vi "Test_INL.vi"(0 "Value":refnum<vi>, 5 "Total":refnum<vi>, 11 "Error In":errorcluster) -> (4 "INL":dbl[](array[numeric]) format="%#.6g", 6 "Codes Array":i32[](array[numeric]), 15 "Error Out":errorcluster)   [LabVIEW 2026, in "Core.lvlib"]
doc: "Calculates INL values and identifies the corresponding converter codes for linearity characterization."
uses:
  Core.lvlib
  TypeDefs/Enum_Notifier_Name.ctl
  TypeDefs/Enum_Notifier_Options.ctl
  TypeDefs/Notification_Clusters/Cluster_INL_Measurement_Specs.ctl
  <instrlib>/niDCPower/nidcpower.llb/niDCPower Output Function.ctl
  TypeDefs/Notification_Clusters/Cluster_ADC_Instrument_Specs.ctl
  TypeDefs/Notification_Clusters/Cluster_DAC_Instrument_Specs.ctl
  <instrlib>/niDCPower/nidcpower.llb/niDCPower Measurement Type.ctl
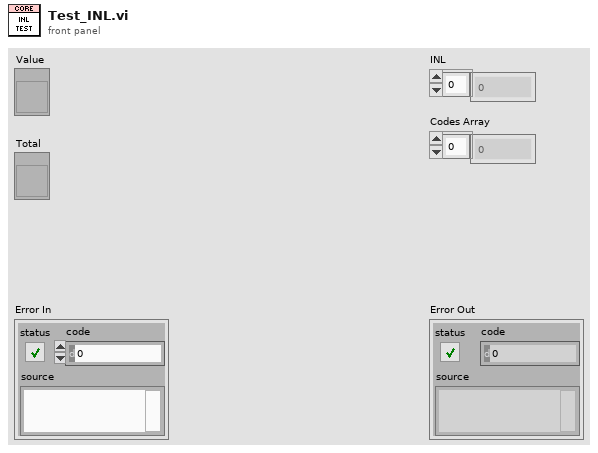
[diagram p1: front panel]
types:
  T1 = typedef "Core.lvlib/Cluster_INL_Measurement_Specs.ctl" = cluster{" Resolution":u16, "Reference Voltage":dbl, "Settling Time (ms)":u32, "Start":dbl, "Step Size":dbl, "Stop":dbl}
  T2 = typedef "Core.lvlib/Enum_Notifier_Options.ctl" = enum16{"Create", "Send", "Status", "Release"}
  T3 = typedef "Core.lvlib/Enum_Notifier_Name.ctl" = enum16{"Device Type", "Test", "Instrument Spec", "Measurement Spec", "Status"}
  T4 = typedef "Core.lvlib/Cluster_ADC_Instrument_Specs.ctl" = cluster{"ADC Source":refnum<k15>, "Current Limit":dbl, "Voltage Level Range":dbl, "ADC DUT":string}
  T5 = typedef "Core.lvlib/Cluster_DAC_Instrument_Specs.ctl" = cluster{"DAC Measurement Device":refnum<k15>, "Current Limit":dbl, "Voltage Level Range":dbl, "DAC DUT":string}
  T6 = typedef "niDCPower Output Function.ctl" = i32
  T7 = typedef "niDCPower Measurement Type.ctl" = i32
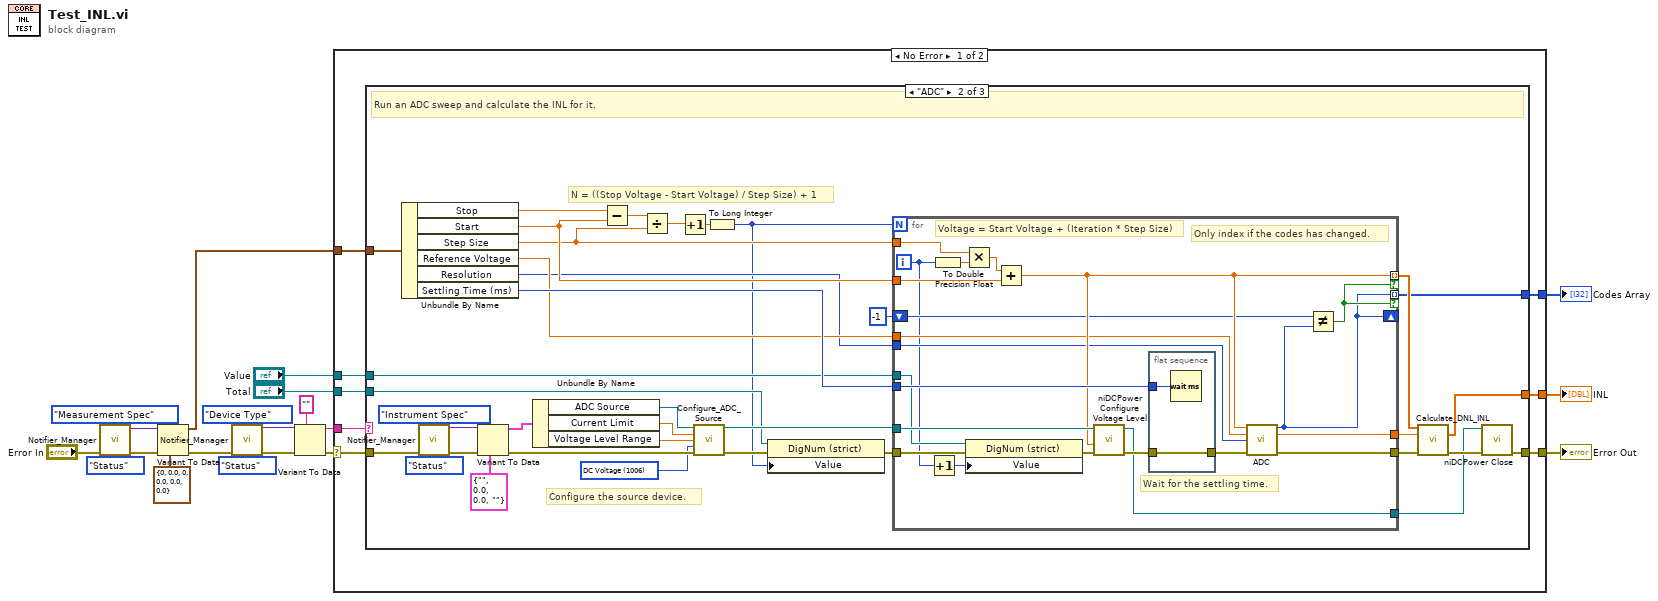
[diagram p0: block diagram]
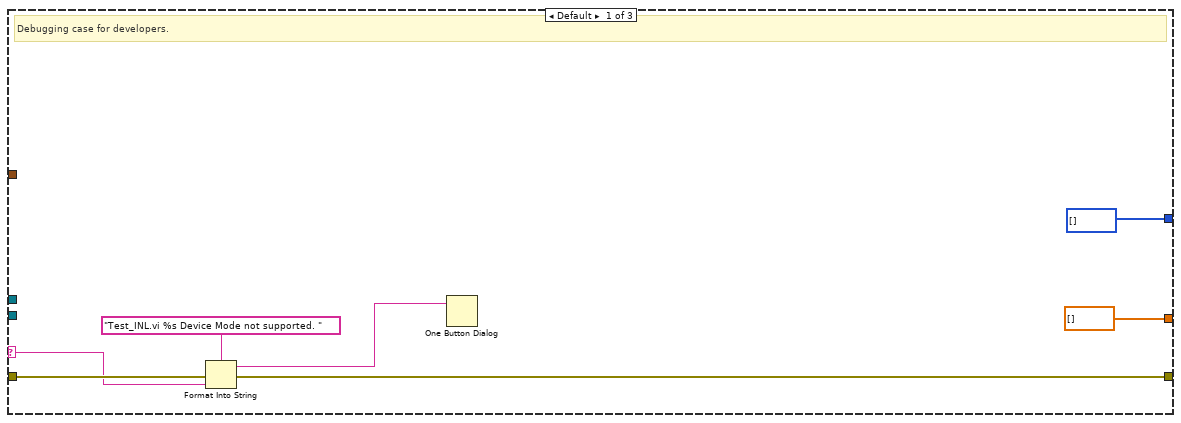
[diagram p2: hidden frame]
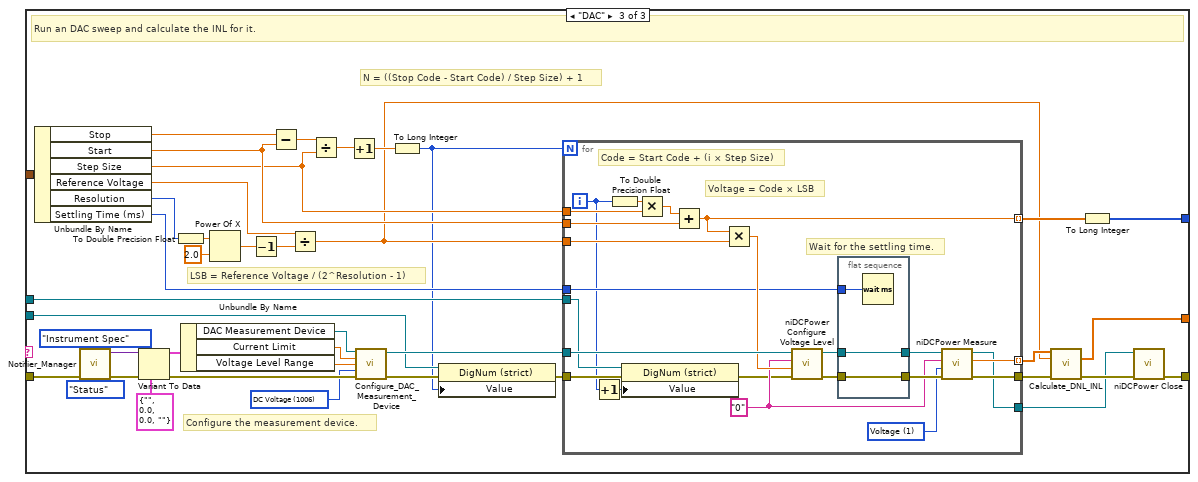
[diagram p3: hidden frame]
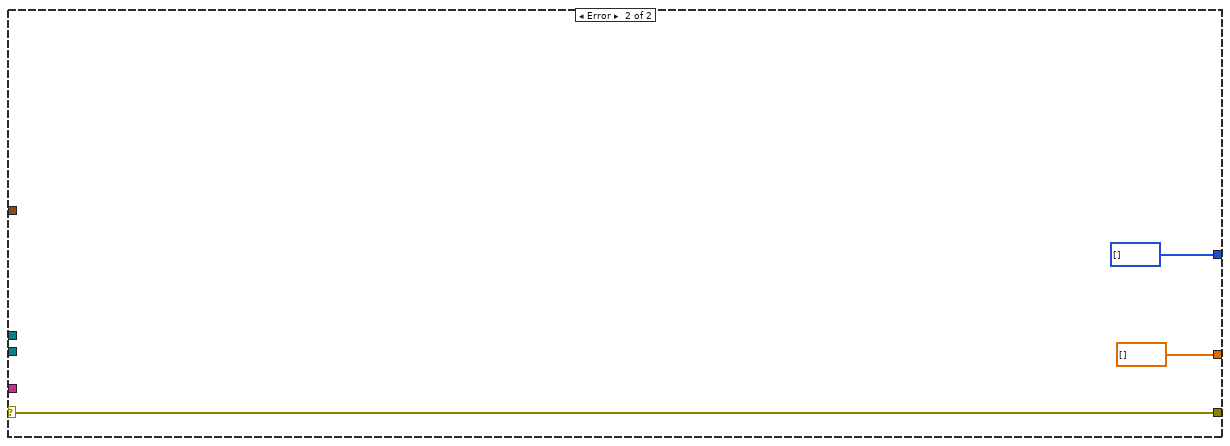
[diagram p4: hidden frame]
diagram:
  n1 = call "Notifier_Manager.vi"("Notifier Name"=Enum_Notifier_Name."Measurement Spec", "Error In"="Error In", "Notifier Options"=Enum_Notifier_Options."Status") -> ("Notifier Data"=w17:variant, "Error Out"=w12:errorcluster)  [unwired: 11 in]
  n2 = Variant To Data(error in=w12, type=T1 {" Resolution"=0, "Reference Voltage"=0.0, "Settling Time (ms)"=0, "Start"=0.0, "Step Size"=0.0, "Stop"=0.0} ("Measurement Specs"), Variant=w17) -> (data=w5:T1, error out=w15:errorcluster)
  n3 = call "Notifier_Manager.vi"("Notifier Name"=Enum_Notifier_Name."Device Type", "Error In"=w15, "Notifier Options"=Enum_Notifier_Options."Status") -> ("Notifier Data"=w10:variant, "Error Out"=w9:errorcluster)  [unwired: 11 in]
  n4 = Variant To Data(error in=w9, type="", Variant=w10) -> (data=w4:string, error out=w6:errorcluster)
  n5 = case shown="No Error" w6 {
    selector: w6 -> [w24 w166]
    tunnel: [w28 w166] -> w20
    tunnel: [w27 dbl[] [] ("INL")] -> w19
    tunnel: [w26 i32[] [] ("INL")] -> w18
    tunnel: w5 -> [w25 _]
    tunnel: w4 -> [w23 _]
    tunnel: "Value" -> [w22 _]
    tunnel: "Total" -> [w21 _]
    frame No Error {
      n6 = case shown="\"ADC\"" w23 {
        selector: w23 -> [w32 _ _]
        tunnel: w24 -> [w35 w70 w137]
        tunnel: [w34 w43 w104] -> w28
        tunnel: w25 -> [_ w54 w130]
        tunnel: [dbl[] [] ("INL") w46 w129] -> w27
        tunnel: [i32[] [] ("INL") w45 w98] -> w26
        tunnel: w22 -> [_ w41 w102]
        tunnel: w21 -> [_ w38 w100]
        frame Default {
          # "Debugging case for developers."
          n7 = Format Into String(format string="Test_INL.vi %s Device Mode not supported. " ("message"), error in=w35, w32) -> (resulting string=w31:string, error out=w34:errorcluster)  [unwired: 1 in]
          n8 = One Button Dialog(message=w31) -> ()  [unwired: 1 in, 1 out]
        }
        frame "ADC" {
          w36 = T6 1006 items=["DC Voltage"=1006, "DC Current"=1007, "Pulse Voltage"=1049, "Pulse Current"=1050, "Constant Resistance"=1161, "Constant Power"=1162] ("output function")
          # "Configure the source device."
          # "N = ((Stop Voltage - Start Voltage) / Step Size) + 1"
          # "Run an ADC sweep and calculate the INL for it."
          n9 = Unbundle By Name(w54) -> ("Stop"=w61:dbl, "Start"=w57:dbl, "Step Size"=w56:dbl, "Reference Voltage"=w52:dbl, "Resolution"=w51:u16, "Settling Time (ms)"=w53:u32)
          n10 = call "Notifier_Manager.vi"("Notifier Name"=Enum_Notifier_Name."Instrument Spec", "Error In"=w70, "Notifier Options"=Enum_Notifier_Options."Status") -> ("Notifier Data"=w65:variant, "Error Out"=w67:errorcluster)  [unwired: 11 in]
          n11 = Variant To Data(error in=w67, type=T4 {"ADC Source"="", "Current Limit"=0.0, "Voltage Level Range"=0.0, "ADC DUT"=""} ("ADC Instrument Spec"), Variant=w65) -> (data=w64:T4, error out=w63:errorcluster)
          n12 = Unbundle By Name(w64) -> ("ADC Source"=w62:refnum<k15>, "Current Limit"=w71:dbl, "Voltage Level Range"=w72:dbl)
          n13 = Subtract(x=w61, y=w57) -> (x-y=w60:dbl)
          n14 = Divide(x=w60, y=w56) -> (x/y=w59:dbl)
          n15 = Increment(x=w59) -> (x+1=w58:dbl)
          n16 = call "Configure_ADC_Source.vi"("Resource Name"=w62, "Current Limit"=w71, "Voltage Level Range"=w72, "Output Function"=w36, "Error In"=w63) -> ("Instrument Handle"=w55:refnum<k15>, "Error Out"=w39:errorcluster)  [unwired: 9 in]
          n17 = To Long Integer(number=w58) -> (32bit integer=w37:i32)
          n18 = property class="DigNum (strict)"(reference=w38, error in=w39, "Value"=w37) -> (error out=w40:errorcluster)  [unwired: 1 out]
          n19 = for {
            N: w37 -> [_]
            tunnel: w40 -> [w90]
            tunnel: w57 -> [w91]
            tunnel: w56 -> [w94]
            tunnel: [w85] -> w49 mode=indexing if=w78
            tunnel: w55 -> [w89]
            tunnel: w53 -> [w86]
            tunnel: w52 -> [w84]
            tunnel: w51 -> [w83]
            tunnel: [w82] -> w48
            tunnel: [w81] -> w42
            shift-right: [w74] -> _
            shift-left: -1 ("Code") -> [w80]
            tunnel: [w79] -> w47
            tunnel: [w74] -> w45 mode=indexing if=w78
            tunnel: w41 -> [w76]
            i -> [w75]
            # "Wait for the settling time."
            # "Only index if the codes has changed."
            # "Voltage = Start Voltage + (Iteration * Step Size)"
            n20 = Increment(x=w75) -> (x+1=w73:i32)
            n21 = To Double Precision Float(number=w75) -> (double precision float=w93:dbl)
            n22 = Multiply(x=w94, y=w93) -> (x*y=w92:dbl)
            n23 = property class="DigNum (strict)"(reference=w76, error in=w90, "Value"=w73) -> (error out=w77:errorcluster)  [unwired: 1 out]
            n24 = Add(x=w92, y=w91) -> (x+y=w85:dbl)
            n25 = call <instrlib>:"niDCPower Configure Voltage Level.vi"("error in (no error)"=w77, "voltage level"=w85, "instrument handle"=w89) -> ("error out"=w88:errorcluster, "instrument handle out"=w81:refnum<k15>)  [unwired: 7 in]
            n26 = flat-sequence {
              tunnel: w88 -> [w96]
              tunnel: [w96] -> w87
              tunnel: w86 -> [w95]
              frame #0 {
                n27 = Wait (ms)(milliseconds to wait=w95) -> ()  [unwired: 1 out]
              }
            }
            n28 = call "ADC.vi"("Input Voltage"=w85, "Reference Voltage"=w84, "Resolution"=w83, "Error In"=w87) -> ("Code"=w74:i32, "LSB"=w79:dbl, "Error Out"=w82:errorcluster)  [unwired: 9 in]
            n29 = Not Equal?(x=w80, y=w74) -> (x != y?=w78:bool)
          }
          n30 = call "Calculate_DNL_INL.vi"("Transition Voltage"=w49, "LSB"=w47, "error in (no error)"=w48) -> ("INL"=w46:dbl[], "error out"=w44:errorcluster)  [unwired: 10 in, 1 out]
          n31 = call <instrlib>:"niDCPower Close.vi"("error in (no error)"=w44, "instrument handle"=w42) -> ("error out"=w43:errorcluster)  [unwired: 9 in]
        }
        frame "DAC" {
          w97 = T6 1006 items=["DC Voltage"=1006, "DC Current"=1007, "Pulse Voltage"=1049, "Pulse Current"=1050, "Constant Resistance"=1161, "Constant Power"=1162] ("Output Function")
          # "Configure the measurement device."
          # "N = ((Stop Code - Start Code) / Step Size) + 1"
          # "LSB = Reference Voltage / (2^Resolution - 1)"
          # "Run an DAC sweep and calculate the INL for it."
          n32 = Unbundle By Name(w130) -> ("Stop"=w119:dbl, "Start"=w118:dbl, "Step Size"=w117:dbl, "Reference Voltage"=w123:dbl, "Resolution"=w124:u16, "Settling Time (ms)"=w108:u32)
          n33 = call "Notifier_Manager.vi"("Notifier Name"=Enum_Notifier_Name."Instrument Spec", "Error In"=w137, "Notifier Options"=Enum_Notifier_Options."Status") -> ("Notifier Data"=w132:variant, "Error Out"=w134:errorcluster)  [unwired: 11 in]
          n34 = Variant To Data(error in=w134, type=T5 {"DAC Measurement Device"="", "Current Limit"=0.0, "Voltage Level Range"=0.0, "DAC DUT"=""} ("DAC Instrument Spec"), Variant=w132) -> (data=w131:T5, error out=w114:errorcluster)
          n35 = To Double Precision Float(number=w124) -> (double precision float=w127:dbl)
          n36 = Unbundle By Name(w131) -> ("DAC Measurement Device"=w112:refnum<k15>, "Current Limit"=w111:dbl, "Voltage Level Range"=w110:dbl)
          n37 = Power Of X(1:2.0 ("x"), 2:w127) -> (0:w126:dbl)
          n38 = Decrement(x=w126) -> (x-1=w125:dbl)
          n39 = Subtract(x=w119, y=w118) -> (x-y=w122:dbl)
          n40 = Divide(x=w123, y=w125) -> (x/y=w106:dbl)
          n41 = Divide(x=w122, y=w117) -> (x/y=w121:dbl)
          n42 = Increment(x=w121) -> (x+1=w120:dbl)
          n43 = call "Configure_DAC_Measurement_Device.vi"("Measurement Device"=w112, "Current Limit"=w111, "Voltage Level Range"=w110, "Output Function"=w97, "Error In"=w114) -> ("Instrument Handle"=w109:refnum<k15>, "Error Out"=w113:errorcluster)  [unwired: 9 in]
          n44 = To Long Integer(number=w120) -> (32bit integer=w99:i32)
          n45 = property class="DigNum (strict)"(reference=w100, error in=w113, "Value"=w99) -> (error out=w101:errorcluster)  [unwired: 1 out]
          n46 = for {
            N: w99 -> [_]
            tunnel: w118 -> [w157]
            tunnel: w117 -> [w160]
            tunnel: w106 -> [w156]
            tunnel: [w155] -> w116 mode=indexing
            tunnel: w101 -> [w154]
            tunnel: [w148] -> w115
            tunnel: w109 -> [w153]
            tunnel: w108 -> [w151]
            tunnel: [w144] -> w107 mode=indexing
            tunnel: [w143] -> w103
            tunnel: w102 -> [w140]
            i -> [w139]
            w142 = "0" ("channel name")
            w145 = T7 1 items=["Current", "Voltage"] ("measurement type")
            # "Wait for the settling time."
            # "Voltage = Code × LSB"
            # "Code = Start Code + (i × Step Size)"
            n47 = Increment(x=w139) -> (x+1=w138:i32)
            n48 = To Double Precision Float(number=w139) -> (double precision float=w159:dbl)
            n49 = property class="DigNum (strict)"(reference=w140, error in=w154, "Value"=w138) -> (error out=w141:errorcluster)  [unwired: 1 out]
            n50 = Multiply(x=w159, y=w160) -> (x*y=w158:dbl)
            n51 = Add(x=w158, y=w157) -> (x+y=w155:dbl)
            n52 = Multiply(x=w155, y=w156) -> (x*y=w152:dbl)
            n53 = call <instrlib>:"niDCPower Configure Voltage Level.vi"("error in (no error)"=w141, "voltage level"=w152, "channel name"=w142, "instrument handle"=w153) -> ("error out"=w150:errorcluster, "instrument handle out"=w147:refnum<k15>)  [unwired: 6 in]
            n54 = flat-sequence {
              tunnel: w151 -> [w163]
              tunnel: w150 -> [w162]
              tunnel: [w162] -> w149
              tunnel: w147 -> [w161]
              tunnel: [w161] -> w146
              frame #0 {
                n55 = Wait (ms)(milliseconds to wait=w163) -> ()  [unwired: 1 out]
              }
            }
            n56 = call <instrlib>:"niDCPower Measure.vi"("error in (no error)"=w149, "measurement type"=w145, "channel name"=w142, "instrument handle"=w146) -> ("error out"=w148:errorcluster, "measurement"=w144:dbl, "instrument handle out"=w143:refnum<k15>)  [unwired: 5 in]
          }
          n57 = call "Calculate_DNL_INL.vi"("Transition Voltage"=w107, "LSB"=w106, "error in (no error)"=w115) -> ("INL"=w129:dbl[], "error out"=w105:errorcluster)  [unwired: 10 in, 1 out]
          n58 = To Long Integer(number=w116) -> (32bit integer=w98:i32[])
          n59 = call <instrlib>:"niDCPower Close.vi"("error in (no error)"=w105, "instrument handle"=w103) -> ("error out"=w104:errorcluster)  [unwired: 9 in]
        }
      }
    }
    frame Error {
    }
  }
  "Error Out" <- w20
  "INL" <- w19
  "Codes Array" <- w18
